vi "SLSC_Engine Get Module Name.vi"(8 "error in (no error)":errorcluster, 10 "compiled.settings":T2={"Name"="", "SLSC Name or IP Address"="", "Slot #"=0, "Reservation Access"=3, "Reservation Group"="", "Configuration Data"={"Properties"={"Boolean Properties"=[], "Double Properties"=[], "I32 Properties"=[], "I64 Properties"=[], "String Properties"=[], "U32 Properties"=[], "U64 Properties"=[]}, "Commands"=[], "Reset Commands"=[], "Apply Values on Deployment"=TRUE, "Apply Reset on Undeployment"=TRUE, "Change Commands"=[]}, "SLSC Get/Read Properties"=[], "SLSC Set/Write Properties"=[], "SLSC Dynamic Commands"=[], "Support Modules"=[]} {"Reservation Access" items=["None"=0, "Read Only"=1, "Read/Write"=3]}, 11 "Item Ref in":T1 format="%.0x") -> (0 "error out":errorcluster, 1 "SLSC Module Name":string, 2 "compiled.settings out":T2={"Name"="", "SLSC Name or IP Address"="", "Slot #"=0, "Reservation Access"=3, "Reservation Group"="", "Configuration Data"={"Properties"={"Boolean Properties"=[], "Double Properties"=[], "I32 Properties"=[], "I64 Properties"=[], "String Properties"=[], "U32 Properties"=[], "U64 Properties"=[]}, "Commands"=[], "Reset Commands"=[], "Apply Values on Deployment"=TRUE, "Apply Reset on Undeployment"=TRUE, "Change Commands"=[]}, "SLSC Get/Read Properties"=[], "SLSC Set/Write Properties"=[], "SLSC Dynamic Commands"=[], "Support Modules"=[]} {"Reservation Access" items=["None"=0, "Read Only"=1, "Read/Write"=3]}, 3 "Item Ref out":T1 format="%.0x")   [LabVIEW 2020, in "SLSC EDS Engine.lvlib"]
uses:
  SLSC EDS Engine.lvlib
  <vilib>/NI VeriStand/Custom Device API/Custom Device API.lvlib
  Shared/SLSC Static Settings.ctl
  Shared/SLSC EDS Shared.lvlib
  SLSC CD API/SLSC CD Engine/SLSC Dynamic Channel.ctl
  SLSC CD API/SLSC CD Shared/SLSC CD Shared.lvlib
  Shared/Compiled.Settings.ctl
  <vilib>/NI VeriStand/Custom Device API/Custom Device Item Ref.ctl
  SLSC CD API/SLSC CD Engine/SLSC Datatype.ctl
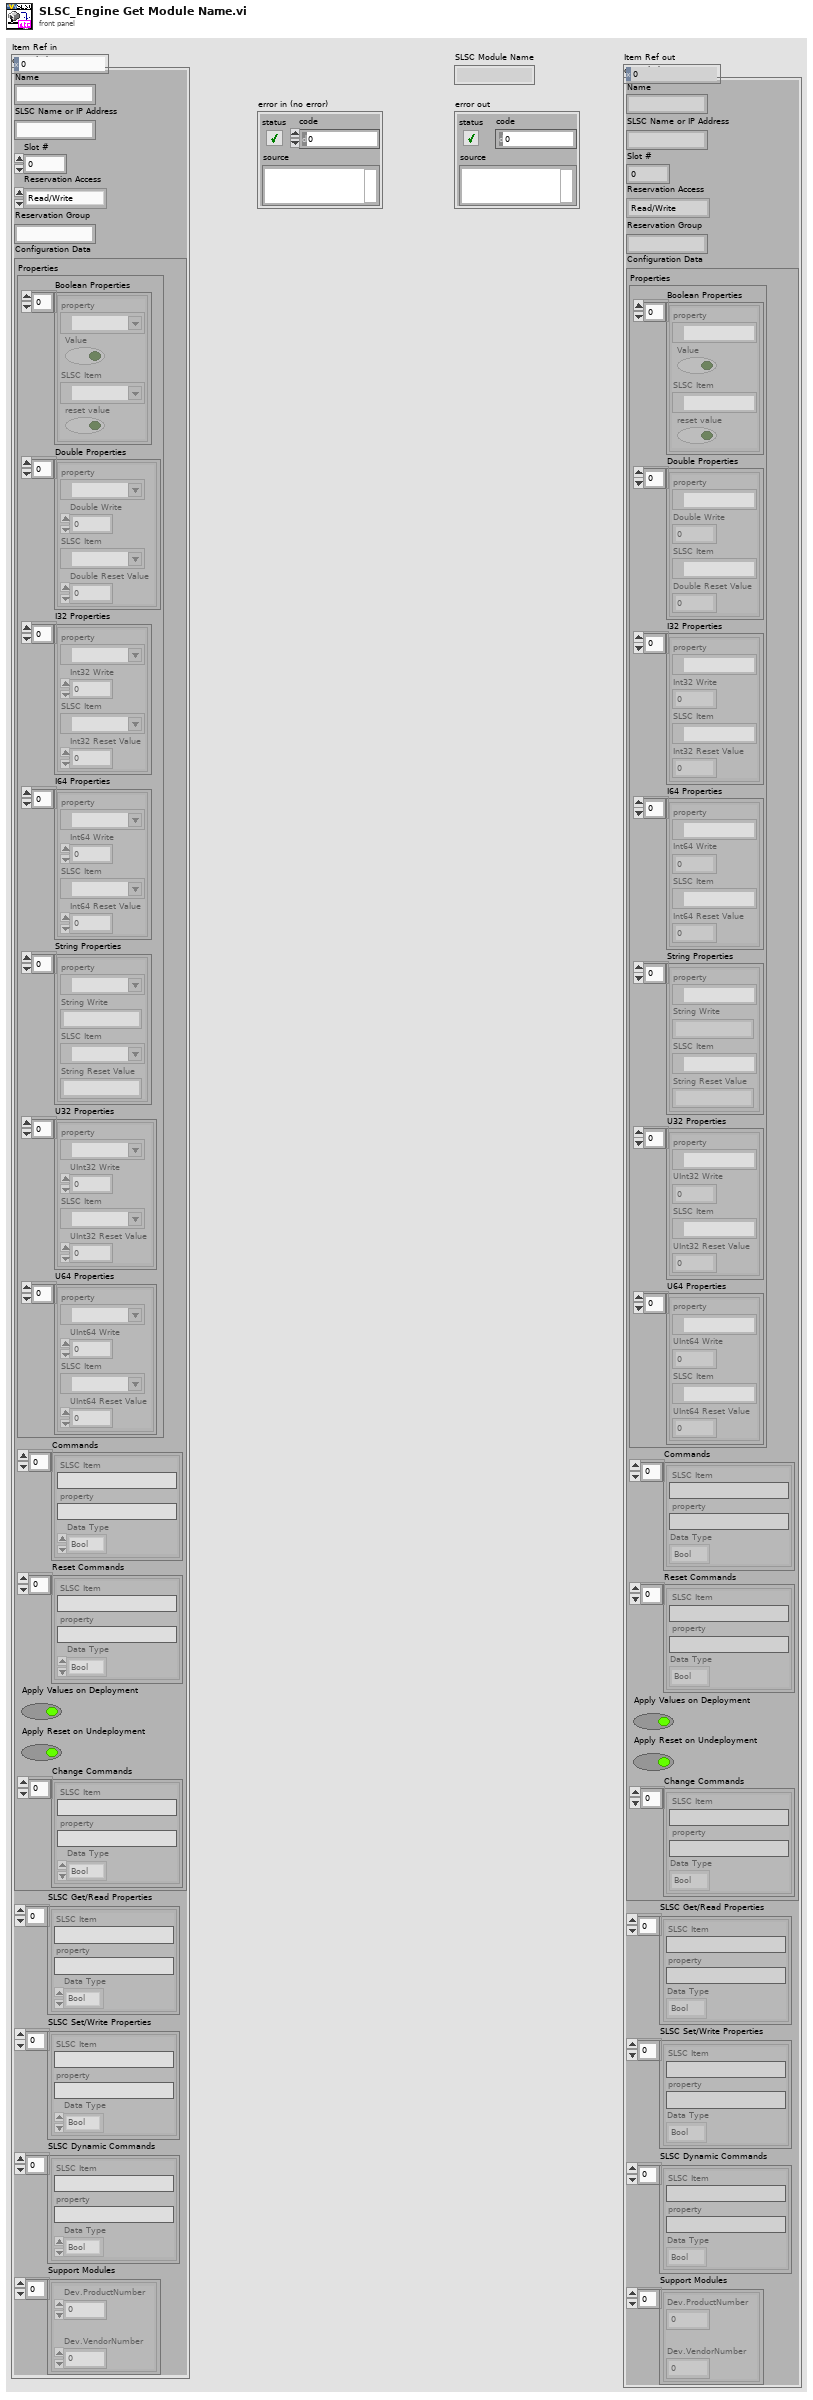
[diagram p1: front panel]
types:
  T1 = typedef "Custom Device API.lvlib/Custom Device Item Ref.ctl" = u64
  T2 = typedef "SLSC EDS Shared.lvlib/Compiled.Settings.ctl" = cluster{"Name":string, "SLSC Name or IP Address":string, "Slot #":i32, "Reservation Access":i32, "Reservation Group":string, "Configuration Data":T3, "SLSC Get/Read Properties":T4[], "SLSC Set/Write Properties":T4[], "SLSC Dynamic Commands":T4[], "Support Modules":cluster{"Dev.ProductNumber":u32, "Dev.VendorNumber":u32}[]}
  T3 = typedef "SLSC EDS Shared.lvlib/SLSC Static Settings.ctl" = cluster{"Properties":cluster{"Boolean Properties":cluster{"property":refnum<k21>, "Value":bool, "SLSC Item":refnum<k21>, "reset value":bool}[], "Double Properties":cluster{"property":refnum<k21>, "Double Write":dbl, "SLSC Item":refnum<k21>, "Double Reset Value":dbl}[], "I32 Properties":cluster{"property":refnum<k21>, "Int32 Write":i32, "SLSC Item":refnum<k21>, "Int32 Reset Value":i32}[], "I64 Properties":cluster{"property":refnum<k21>, "Int64 Write":i64, "SLSC Item":refnum<k21>, "Int64 Reset Value":i64}[], "String Properties":cluster{"property":refnum<k21>, "String Write":string, "SLSC Item":refnum<k21>, "String Reset Value":string}[], "U32 Properties":cluster{"property":refnum<k21>, "UInt32 Write":u32, "SLSC Item":refnum<k21>, "UInt32 Reset Value":u32}[], "U64 Properties":cluster{"property":refnum<k21>, "UInt64 Write":u64, "SLSC Item":refnum<k21>, "UInt64 Reset Value":u64}[]}, "Commands":T4[], "Reset Commands":T4[], "Apply Values on Deployment":bool, "Apply Reset on Undeployment":bool, "Change Commands":T4[]}
  T4 = typedef "SLSC CD Shared.lvlib/SLSC Dynamic Channel.ctl" = cluster{"SLSC Item":string, "property":string, "Data Type":T5}
  T5 = typedef "SLSC CD Shared.lvlib/SLSC Datatype.ctl" = enum16{"Bool", "Double", "I32", "I64", "String", "U32", "U64"}
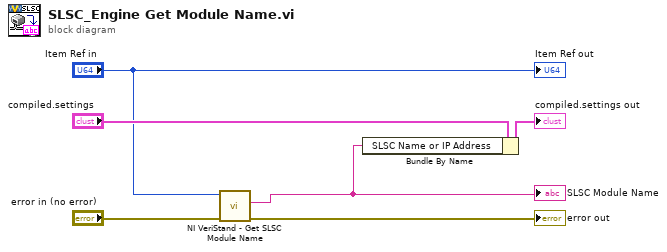
[diagram p0: block diagram]
diagram:
  n1 = call <vilib>:"NI VeriStand - Get SLSC Module Name.vi"("error in (no error)"="error in (no error)", "Item Ref in"="Item Ref in") -> ("error out"=→"error out":errorcluster, "SLSC Module"=w2:string)  [unwired: 7 in, 1 out]
  "SLSC Module Name" <- w2
  n2 = Bundle By Name(cluster="compiled.settings", "SLSC Name or IP Address"=w2) -> (→"compiled.settings out":T2)
  "Item Ref out" <- "Item Ref in"
